vi "1d.amplitude_and_pixels.vi"() -> ()   [LabVIEW 2017]
uses:
  <vilib>/Instr/_visa.llb/VISA Configure Serial Port (Instr).vi
panel:
  out "XY Graph":cluster{dbl[], u16[]}(graph)
  out "appended array":dbl[][](array[numeric])
  out "size(s) 2":i32
  out "appended array 2":dbl[](array[numeric])
  out "size(s)":i32
  out "Waveform Graph":u16[](graph)
  out "array w/ subset deleted":u16[](array[numeric])
  out "byte swapped":u16[](array[numeric])
  out "*(type *) &x":u16[](array[numeric])
  out "substring":string
  out "x-y":i32
  out "length":i32
  in  "Integration time (µs) 2":i32=100000
  out "read buffer 3":string
  out "read buffer 2":string
  out "VISA resource name out":refnum<visa-resource-name>
  out "read buffer":string
  in  "VISA resource name":refnum<visa-resource-name>="COM3" caption="Serial COM port"
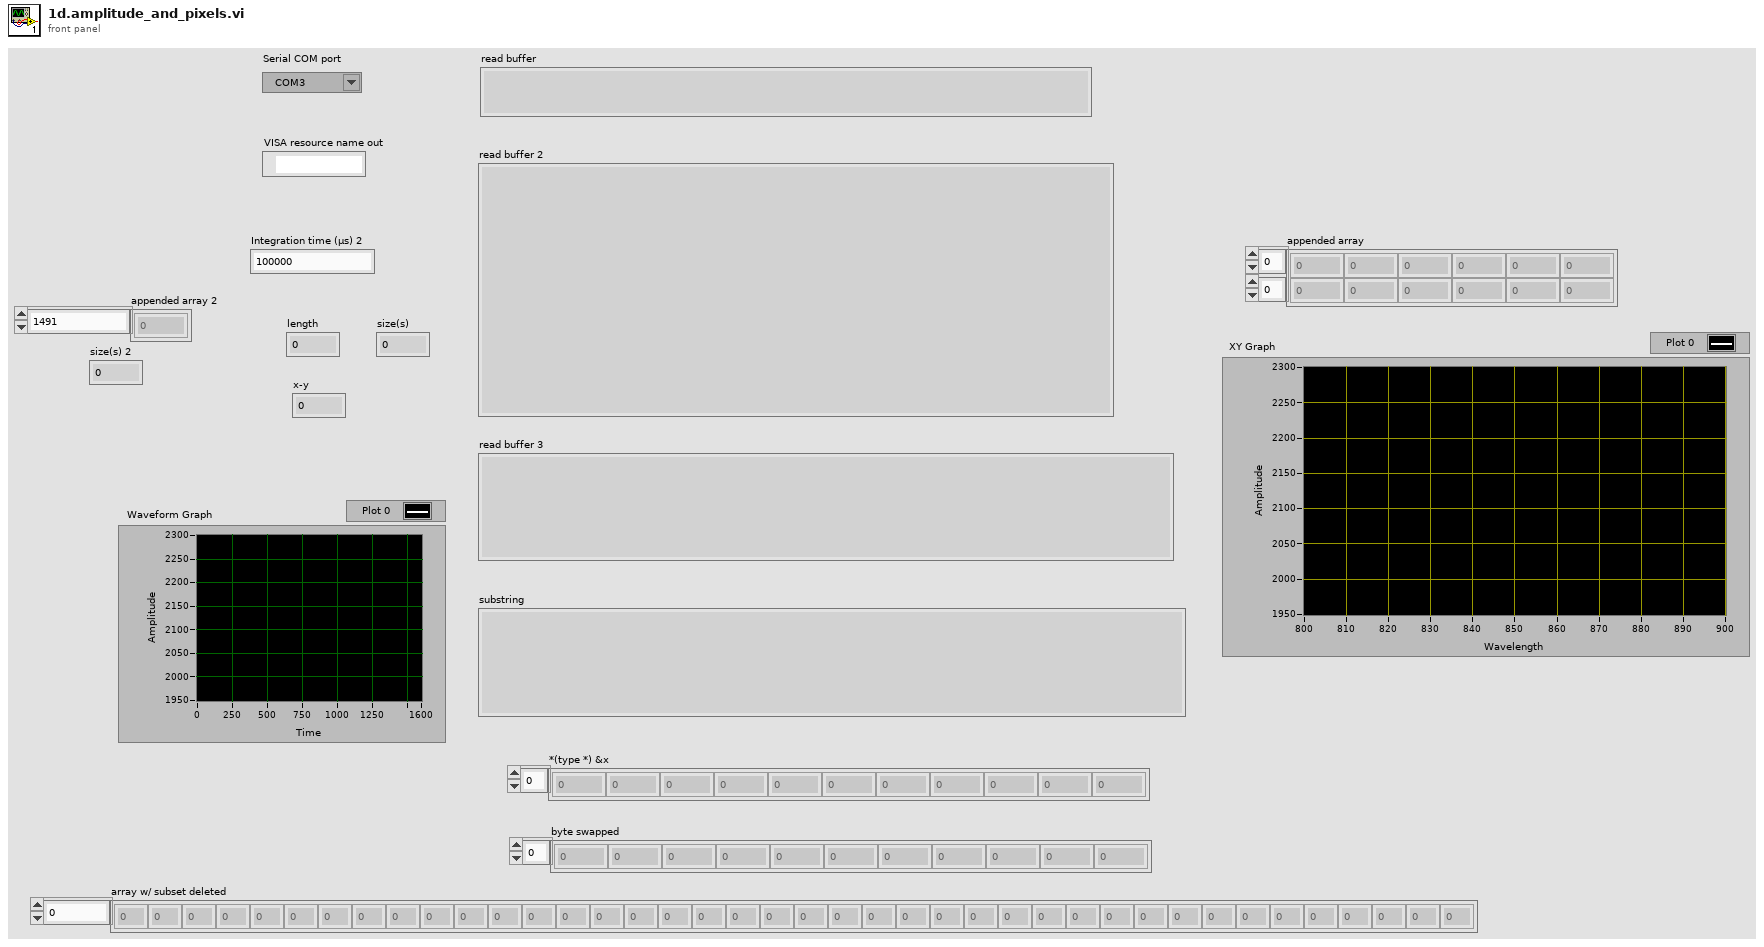
[diagram p1: front panel]
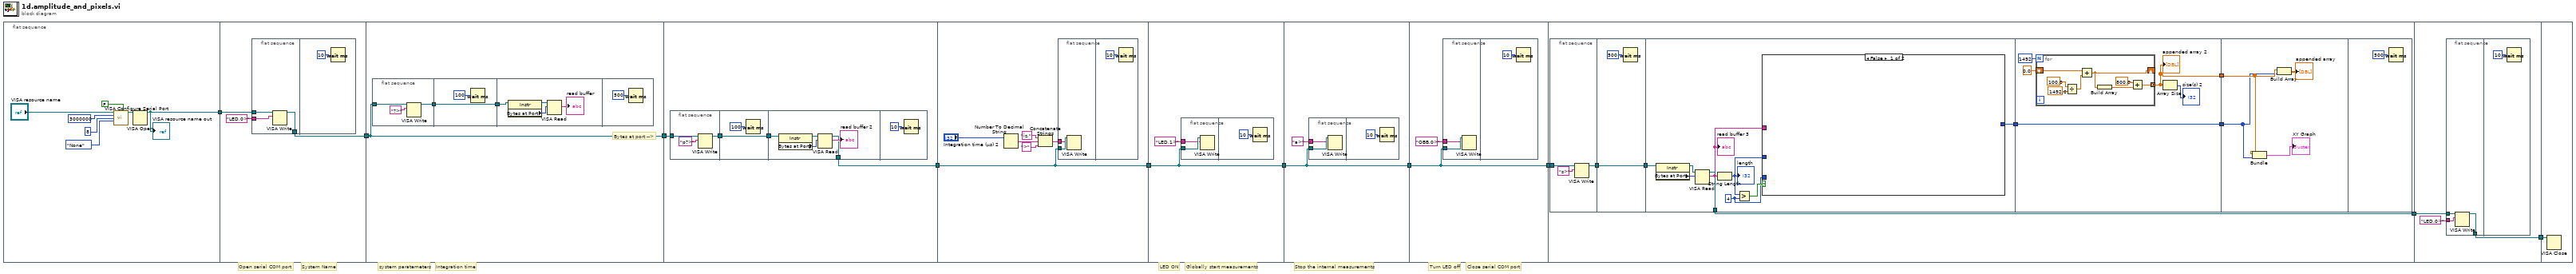
[diagram p0: block diagram]
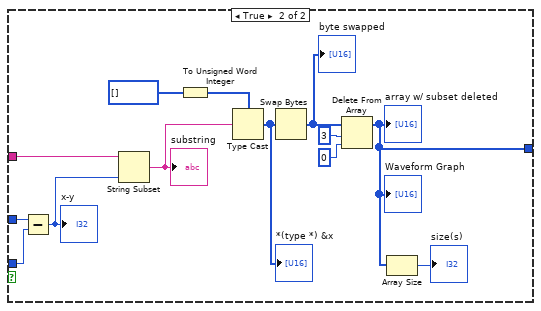
[diagram p2: hidden frame]
diagram:
  # "Globally start measurements"
  # "LED ON"
  # "System Name"
  # "Integration time"
  # "system paratemeters"
  # "Close serial COM port"
  # "Turn LED off"
  # "Stop the internal measurements"
  # "Open serial COM port"
  n1 = flat-sequence {
    tunnel: [w13] -> w3
    tunnel: w3 -> [w19]
    tunnel: [w18] -> w2
    tunnel: w2 -> [w25]
    tunnel: [w25] -> w10
    tunnel: w10 -> [w39]
    tunnel: [w38] -> w9
    tunnel: w9 -> [w53]
    tunnel: [w53] -> w8
    tunnel: w8 -> [w62]
    tunnel: [w62] -> w1
    tunnel: [w67] -> w7
    tunnel: w1 -> [w67]
    tunnel: w7 -> [w72]
    tunnel: [w72] -> w6
    tunnel: w6 -> [w81]
    tunnel: [w80] -> w5
    tunnel: w5 -> [w130]
    tunnel: [w129] -> w4
    tunnel: w4 -> [w136]
    frame #0 {
      n2 = call-poly "VISA Configure Serial Port"("VISA resource name"="VISA resource name", "Enable Termination\nChar (T)"=FALSE ("Enable Termination\nChar (T)"), "baud rate (9600)"=u32 3000000, "data bits (8)"=u16 8, "parity (0:none)"=enum16{"None", "Odd", "Even", "Mark", "Space"}."None") -> ("VISA resource name out"=w17:refnum<visa-resource-name>)  [unwired: 9 in, 1 out]
      n3 = VISA Open(VISA resource name=w17) -> (VISA resource name=w13:refnum<visa-resource-name>)  [unwired: 4 in, 1 out]
      "VISA resource name out" <- w13
    }
    frame #1 {
      n4 = flat-sequence {
        tunnel: w19 -> [w23]
        tunnel: "LED,0>" ("String") -> [w22]
        tunnel: [w21] -> w18
        frame #0 {
          n5 = VISA Write(VISA resource name=w23, write buffer=w22) -> (VISA resource name out=w21:refnum<visa-resource-name>)  [unwired: 1 in, 2 out]
        }
        frame #1 {
          n6 = Wait (ms)(milliseconds to wait=u32 10 ("Zu wartende ms")) -> ()  [unwired: 1 out]
        }
      }
    }
    frame #2 {
      # "Bytes at port -->"
      n7 = flat-sequence {
        tunnel: [w30] -> w27
        tunnel: w25 -> [w29]
        tunnel: [w31] -> w26
        tunnel: w27 -> [w31]
        tunnel: w26 -> [w36]
        frame #0 {
          n8 = VISA Write(VISA resource name=w29, write buffer="?>") -> (VISA resource name out=w30:refnum<visa-resource-name>)  [unwired: 1 in, 2 out]
        }
        frame #1 {
          n9 = Wait (ms)(milliseconds to wait=u32 100 ("Zu wartende ms")) -> ()  [unwired: 1 out]
        }
        frame #2 {
          n10 = property class="Instr"(reference=w36) -> (reference out=w35:refnum<visa-resource-name>, "Bytes at Port"=w34:u32)  [unwired: 1 in, 1 out]
          n11 = VISA Read(VISA resource name=w35, byte count=w34) -> (read buffer=→"read buffer":string)  [unwired: 1 in, 3 out]
        }
        frame #3 {
          n12 = Wait (ms)(milliseconds to wait=u32 500 ("Zu wartende ms")) -> ()  [unwired: 1 out]
        }
      }
    }
    frame #3 {
      n13 = flat-sequence {
        tunnel: [w44] -> w41
        tunnel: w39 -> [w42]
        tunnel: [w45] -> w40
        tunnel: w41 -> [w45]
        tunnel: w40 -> [w51]
        tunnel: [w47] -> w38
        frame #0 {
          n14 = VISA Write(VISA resource name=w42, write buffer="p?>") -> (VISA resource name out=w44:refnum<visa-resource-name>)  [unwired: 1 in, 2 out]
        }
        frame #1 {
          n15 = Wait (ms)(milliseconds to wait=u32 100 ("Zu wartende ms")) -> ()  [unwired: 1 out]
        }
        frame #2 {
          n16 = property class="Instr"(reference=w51) -> (reference out=w50:refnum<visa-resource-name>, "Bytes at Port"=w49:u32)  [unwired: 1 in, 1 out]
          n17 = VISA Read(VISA resource name=w50, byte count=w49) -> (VISA resource name out=w47:refnum<visa-resource-name>, read buffer=→"read buffer 2":string)  [unwired: 1 in, 2 out]
        }
        frame #3 {
          n18 = Wait (ms)(milliseconds to wait=u32 10 ("Zu wartende ms")) -> ()  [unwired: 1 out]
        }
      }
    }
    frame #4 {
      n19 = Number To Decimal String(number="Integration time (µs) 2") -> (decimal integer string=w58:string)  [unwired: 1 in]
      n20 = Concatenate Strings("iz," ("String"), w58, ">" ("String")) -> (w55:string)
      n21 = flat-sequence {
        tunnel: w53 -> [w60]
        tunnel: w55 -> [w59]
        frame #0 {
          n22 = VISA Write(VISA resource name=w60, write buffer=w59) -> ()  [unwired: 1 in, 3 out]
        }
        frame #1 {
          n23 = Wait (ms)(milliseconds to wait=u32 10 ("Zu wartende ms")) -> ()  [unwired: 1 out]
        }
      }
    }
    frame #5 {
      n24 = flat-sequence {
        tunnel: w62 -> [w65]
        tunnel: "LED,1>" ("String") -> [w64]
        frame #0 {
          n25 = VISA Write(VISA resource name=w65, write buffer=w64) -> ()  [unwired: 1 in, 3 out]
        }
        frame #1 {
          n26 = Wait (ms)(milliseconds to wait=u32 10 ("Zu wartende ms")) -> ()  [unwired: 1 out]
        }
      }
    }
    frame #6 {
      n27 = flat-sequence {
        tunnel: w67 -> [w70]
        tunnel: "a>" ("String") -> [w69]
        frame #0 {
          n28 = VISA Write(VISA resource name=w70, write buffer=w69) -> ()  [unwired: 1 in, 3 out]
        }
        frame #1 {
          n29 = Wait (ms)(milliseconds to wait=u32 10 ("Zu wartende ms")) -> ()  [unwired: 1 out]
        }
      }
    }
    frame #7 {
      n30 = flat-sequence {
        tunnel: w72 -> [w75]
        tunnel: "OBB,0>" ("String") -> [w74]
        frame #0 {
          n31 = VISA Write(VISA resource name=w75, write buffer=w74) -> ()  [unwired: 1 in, 3 out]
        }
        frame #1 {
          n32 = Wait (ms)(milliseconds to wait=u32 10 ("Zu wartende ms")) -> ()  [unwired: 1 out]
        }
      }
    }
    frame #8 {
      n33 = flat-sequence {
        tunnel: [w86] -> w83
        tunnel: w81 -> [w84]
        tunnel: [w87] -> w82
        tunnel: w83 -> [w87]
        tunnel: w82 -> [w97]
        tunnel: [w96] -> w80
        tunnel: [w89] -> w77
        tunnel: [w112] -> w79
        tunnel: [w111] -> w78
        tunnel: w77 -> [w111]
        tunnel: w79 -> [w126]
        tunnel: w78 -> [w125]
        frame #0 {
          n34 = VISA Write(VISA resource name=w84, write buffer="s>") -> (VISA resource name out=w86:refnum<visa-resource-name>)  [unwired: 1 in, 2 out]
        }
        frame #1 {
          n35 = Wait (ms)(milliseconds to wait=u32 500 ("Zu wartende ms")) -> ()  [unwired: 1 out]
        }
        frame #2 {
          w90 = 4 ("y")
          n36 = property class="Instr"(reference=w97) -> (reference out=w95:refnum<visa-resource-name>, "Bytes at Port"=w94:u32)  [unwired: 1 in, 1 out]
          n37 = VISA Read(VISA resource name=w95, byte count=w94) -> (VISA resource name out=w96:refnum<visa-resource-name>, read buffer=w93:string)  [unwired: 1 in, 2 out]
          "read buffer 3" <- w93
          n38 = String Length(string=w93) -> (length=w92:i32)
          "length" <- w92
          n39 = Greater?(x=w92, y=w90) -> (0:w91:bool)
          n40 = case shown="False" w91 {
            tunnel: w93 -> [_ w110]
            tunnel: w92 -> [_ w109]
            tunnel: w90 -> [_ w108]
            tunnel: [_ w98] -> w89
            frame False {
            }
            frame True {
              n41 = Subtract(x=w109, y=w108) -> (x-y=w107:i32)
              "x-y" <- w107
              n42 = String Subset(string=w110, length (rest)=w107) -> (substring=w105:string)  [unwired: 1 in]
              "substring" <- w105
              n43 = To Unsigned Word Integer(number=i32[] []) -> (unsigned 16bit integer=w106:u16[])
              n44 = Type Cast(type=w106, x=w105) -> (*(type *) &x=w103:u16[])
              "*(type *) &x" <- w103
              n45 = Swap Bytes(anything=w103) -> (byte swapped=w102:u16[])
              "byte swapped" <- w102
              n46 = Delete From Array(array=w102, length=3, index=0) -> (array with subset deleted=w98:u16[])  [unwired: 1 out]
              "array w/ subset deleted" <- w98
              "Waveform Graph" <- w98
              n47 = Array Size(array=w98) -> (size(s)=→"size(s)":i32)
            }
          }
        }
        frame #3 {
          n48 = for {
            N: 1492 -> [_]
            shift-right: [w122] -> _
            shift-left: 0.0 -> [w123]
            tunnel: [w119] -> w112 mode=concatenating
            n49 = Divide(x=100.0 ("x/y"), y=1492.0) -> (x/y=w116:dbl)
            n50 = Add(x=w123, y=w116) -> (x+y=w122:dbl)
            n51 = Build Array(w122) -> (w120:dbl[])
            n52 = Add(x=800.0 ("x+y"), y=w120) -> (x+y=w119:dbl[])
          }
          "appended array 2" <- w112
          n53 = Array Size(array=w112) -> (size(s)=→"size(s) 2":i32)
        }
        frame #4 {
          n54 = Bundle(w126, w125) -> (→"XY Graph":cluster{dbl[], u16[]})  [unwired: 1 in]
          n55 = Build Array(w126, w125) -> (→"appended array":dbl[][])
        }
        frame #5 {
          n56 = Wait (ms)(milliseconds to wait=u32 500 ("Zu wartende ms")) -> ()  [unwired: 1 out]
        }
      }
    }
    frame #9 {
      n57 = flat-sequence {
        tunnel: w130 -> [w134]
        tunnel: "LED,0>" ("String") -> [w133]
        tunnel: [w132] -> w129
        frame #0 {
          n58 = VISA Write(VISA resource name=w134, write buffer=w133) -> (VISA resource name out=w132:refnum<visa-resource-name>)  [unwired: 1 in, 2 out]
        }
        frame #1 {
          n59 = Wait (ms)(milliseconds to wait=u32 10 ("Zu wartende ms")) -> ()  [unwired: 1 out]
        }
      }
    }
    frame #10 {
      n60 = VISA Close(VISA resource name=w136) -> ()  [unwired: 1 in, 1 out]
    }
  }
